vi "VIH HelpGen - Build Type Name for Terminal Image File.vi"(11 "variant":variant) -> (1 "Error Cluster":bool, 3 "Name":string)   [LabVIEW 2014]
doc: "::: VI Helpeks :::\nCopyright (c) 2000-2026 Konstantin Shifershteyn. All rights reserved."
panel:
  # "VI Helpeks\nCopyright (c) 2012-2026 Konstantin Shifershteyn"
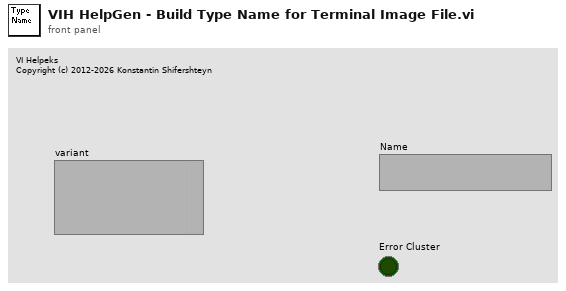
[diagram p1: front panel]
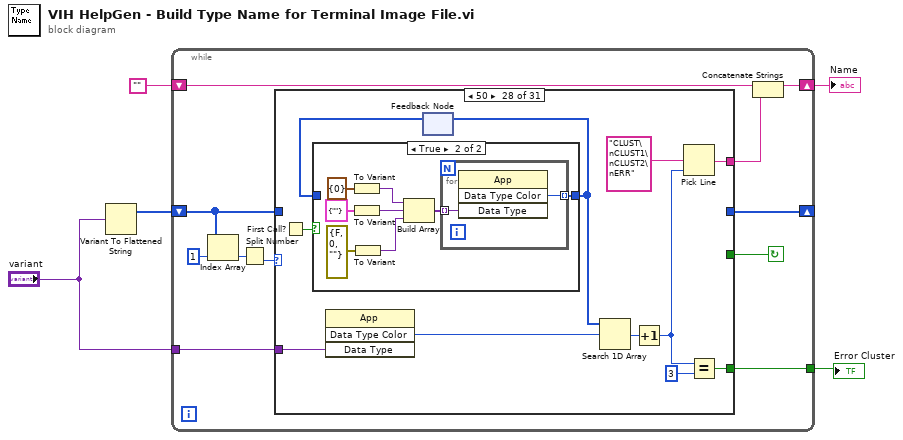
[diagram p0: block diagram]
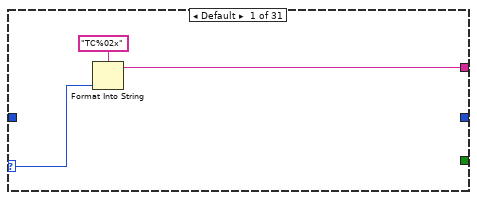
[diagram p2: hidden frame]
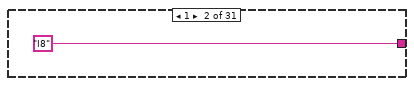
[diagram p3: hidden frame]
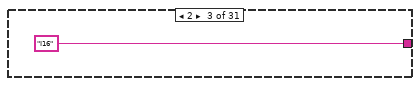
[diagram p4: hidden frame]
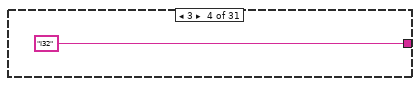
[diagram p5: hidden frame]
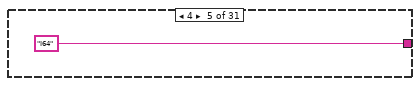
[diagram p6: hidden frame]
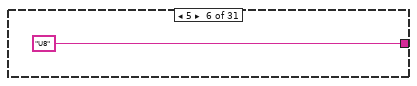
[diagram p7: hidden frame]
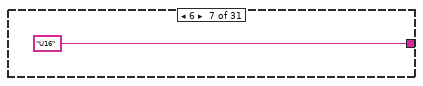
[diagram p8: hidden frame]
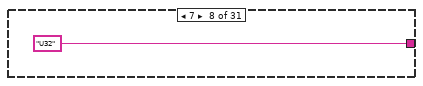
[diagram p9: hidden frame]
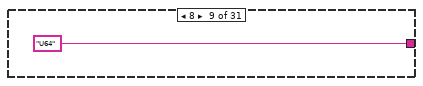
[diagram p10: hidden frame]
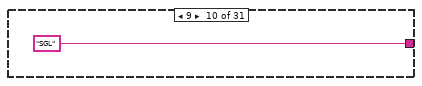
[diagram p11: hidden frame]
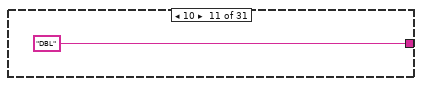
[diagram p12: hidden frame]
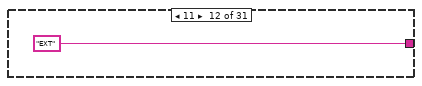
[diagram p13: hidden frame]
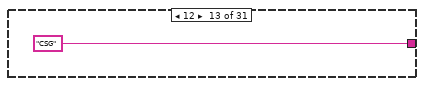
[diagram p14: hidden frame]
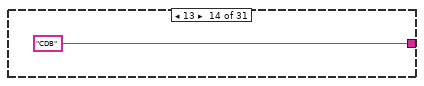
[diagram p15: hidden frame]
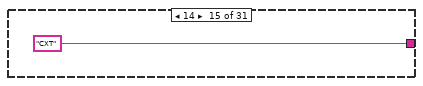
[diagram p16: hidden frame]
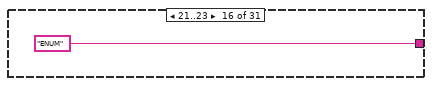
[diagram p17: hidden frame]
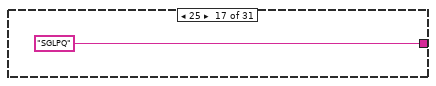
[diagram p18: hidden frame]
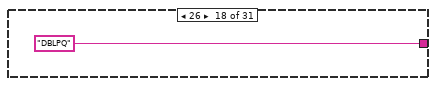
[diagram p19: hidden frame]
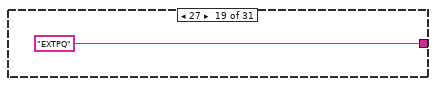
[diagram p20: hidden frame]
diagram:
  n1 = Variant To Flattened String(Variant="variant") -> (1:w5:i16[])  [unwired: 1 out]
  n2 = while {
    shift-right: [w9] -> _
    shift-left: w5 -> [w13]
    shift-right: [w11] -> w3
    shift-left: "" -> [w12]
    tunnel: "variant" -> [w7]
    tunnel: [w6] -> w1
    stop <- w8 continue-if-true
    n3 = Index Array(array=w13, index=1) -> (element=w15:i16)
    n4 = Split Number(x=w15) -> (lo(x)=w14:u8)  [unwired: 1 out]
    n5 = case shown="50" w14 {
      selector: w14 -> [w18 _ _ _ _ _ _ _ _ _ _ _ _ _ _ _ _ _ _ _ _ _ _ _ _ _ _ _ _ _ _]
      tunnel: [w17 "I8" "I16" "I32" "I64" "U8" "U16" "U32" "U64" "SGL" "DBL" "EXT" "CSG" "CDB" "CXT" "ENUM" "SGLPQ" "DBLPQ" "EXTPQ" "CSGPQ" "CDBPQ" "CXTPQ" "BOOL" "STR" "PATH" "PICT" "ARR_" w59 "VAR" w81 "REF"] -> w10
      tunnel: w13 -> [_ _ _ _ _ _ _ _ _ _ _ _ _ _ _ _ _ _ _ _ _ _ _ _ _ _ w48 _ _ w79 _]
      tunnel: [_ _ _ _ _ _ _ _ _ _ _ _ _ _ _ _ _ _ _ _ _ _ _ _ _ _ w46 _ _ _ _] -> w9
      tunnel: [_ _ _ _ _ _ _ _ _ _ _ _ _ _ _ _ _ _ _ _ _ _ _ _ _ _ TRUE _ _ _ _] -> w8
      tunnel: w7 -> [_ _ _ _ _ _ _ _ _ _ _ _ _ _ _ _ _ _ _ _ _ _ _ _ _ _ _ w63 _ _ _]
      tunnel: [_ _ _ _ _ _ _ _ _ _ _ _ _ _ _ _ _ _ _ _ _ _ _ _ _ _ _ w55 _ _ _] -> w6
      frame Default {
        n6 = Format Into String(format string="TC%02x", w18) -> (resulting string=w17:string)  [unwired: 2 in, 1 out]
      }
      frame 1 {
      }
      frame 2 {
      }
      frame 3 {
      }
      frame 4 {
      }
      frame 5 {
      }
      frame 6 {
      }
      frame 7 {
      }
      frame 8 {
      }
      frame 9 {
      }
      frame 10 {
      }
      frame 11 {
      }
      frame 12 {
      }
      frame 13 {
      }
      frame 14 {
      }
      frame 21..23 {
      }
      frame 25 {
      }
      frame 26 {
      }
      frame 27 {
      }
      frame 28 {
      }
      frame 29 {
      }
      frame 30 {
      }
      frame 33 {
      }
      frame 48 {
      }
      frame 50 {
      }
      frame 51 {
      }
      frame 64 {
        n7 = Index Array(array=w48, index=2) -> (element=w52:i16)
        n8 = Multiply(x=w52, y=i16 2) -> (x*y=w50:i16)
        n9 = Add(x=w50, y=i16 3) -> (x+y=w47:i16)
        n10 = Array Subset(array=w48, index=w47) -> (w46:i16[])  [unwired: 1 in]
      }
      frame 80 {
        n11 = First Call?() -> (First Call?: T/F=w64:bool)
        n12 = invoke class="App" method="Data Type Color"("Data Type"=w63) -> ("Data Type Color"=w62:u32)  [unwired: 3 in, 3 out]
        n13 = feedback #1() -> (w65:u32[])  [unwired: 1 in]
        n14 = case shown="True" w64 {
          tunnel: [w66 w69] -> w61
          tunnel: w65 -> [w66 _]
          frame False {
          }
          frame True {
            n15 = To Variant(anything=cluster{i32} {0}) -> (Variant=w72:variant)
            n16 = To Variant(anything=cluster{string} {""}) -> (Variant=w71:variant)
            n17 = To Variant(anything=errorcluster {"status"=FALSE, "code"=0, "source"=""} ("error out")) -> (Variant=w67:variant)
            n18 = Build Array(w72, w71, w67) -> (w70:variant[])
            n19 = for {
              tunnel: w70 -> [w76] mode=indexing
              tunnel: [w75] -> w69 mode=indexing
              n20 = invoke class="App" method="Data Type Color"("Data Type"=w76) -> ("Data Type Color"=w75:u32)  [unwired: 3 in, 3 out]
            }
          }
        }
        n21 = feedback-in #1(w61) -> ()
        n22 = Search 1D Array(1D array=w61, element=w62) -> (index of element=w60:i32)  [unwired: 1 in]
        n23 = Increment(x=w60) -> (x+1=w57:i32)
        n24 = Pick Line(multi-line string="CLUST\nCLUST1\nCLUST2\nERR", line index=w57) -> (output string=w59:string)  [unwired: 1 in]
        n25 = Equal?(x=w57, y=3) -> (x = y?=w55:bool)
      }
      frame 83 {
      }
      frame 84 {
        n26 = Index Array(array=w79, index=2) -> (element=w78:i16)
        n27 = case shown="8" w78 {
          tunnel: ["WFMA" "TS" "WFMD"] -> w81
          frame Default {
          }
          frame 6 {
          }
          frame 8 {
          }
        }
      }
      frame 112 {
      }
    }
    n28 = Concatenate Strings(w12, w10) -> (w11:string)
  }
  "Name" <- w3
  "Error Cluster" <- w1
